vi "UI_Header_Layout.vi"(11 "error in":errorcluster) -> (4 "Specs":T1(array[cluster]), 15 "error out":errorcluster)   [LabVIEW 2026]
doc: "상단 버튼: 0 설정, 1 측정 시작, 2 측정 정지, 3 데이터 저장(저장 중이면 빨강), 4 그래프 창, 5 종료."
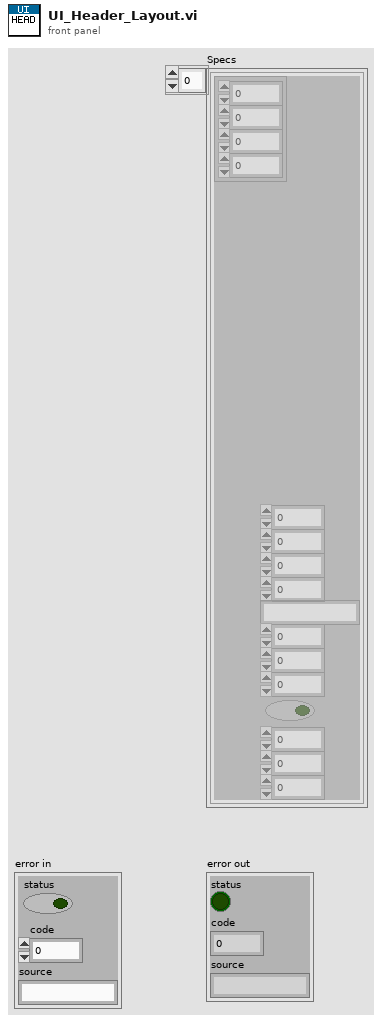
[diagram p1: front panel]
types:
  T1 = cluster{"Rect":cluster{"left":i16, "top":i16, "right":i16, "bottom":i16}, "Fill":u32, "Fill Sel":u32, "Border":u32, "Border Sel":u32, "Text":string, "Text Color":u32, "Text Sel":u32, "Size":i16, "Bold":bool, "Group":i32, "Value":i32, "Radius":i16}[]
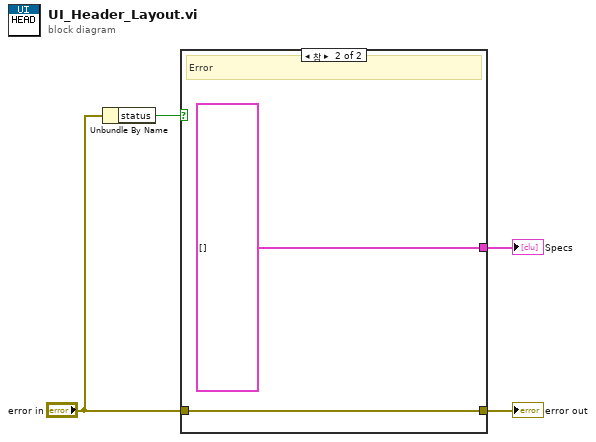
[diagram p0: block diagram]
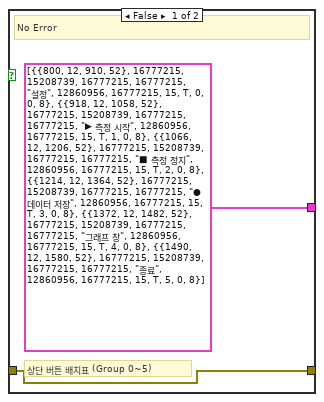
[diagram p2: hidden frame]
diagram:
  n1 = Unbundle By Name("error in") -> ("status"=w2:bool)
  n2 = case shown="참" w2 {
    tunnel: "error in" -> [w5 w7]
    tunnel: [T1 [{"Rect"={"left"=800, "top"=12, "right"=910, "bottom"=52}, "Fill"=16777215, "Fill Sel"=15208739, "Border"=16777215, "Border Sel"=16777215, "Text"="설정", "Text Color"=12860956, "Text Sel"=16777215, "Size"=15, "Bold"=TRUE, "Group"=0, "Value"=0, "Radius"=8}, {"Rect"={"left"=918, "top"=12, "right"=1058, "bottom"=52}, "Fill"=16777215, "Fill Sel"=15208739, "Border"=16777215, "Border Sel"=16777215, "Text"="▶ 측정 시작", "Text Color"=12860956, "Text Sel"=16777215, "Size"=15, "Bold"=TRUE, "Group"=1, "Value"=0, "Radius"=8}, {"Rect"={"left"=1066, "top"=12, "right"=1206, "bottom"=52}, "Fill"=16777215, "Fill Sel"=15208739, "Border"=16777215, "Border Sel"=16777215, "Text"="■ 측정 정지", "Text Color"=12860956, "Text Sel"=16777215, "Size"=15, "Bold"=TRUE, "Group"=2, "Value"=0, "Radius"=8}, {"Rect"={"left"=1214, "top"=12, "right"=1364, "bottom"=52}, "Fill"=16777215, "Fill Sel"=15208739, "Border"=16777215, "Border Sel"=16777215, "Text"="● 데이터 저장", "Text Color"=12860956, "Text Sel"=16777215, "Size"=15, "Bold"=TRUE, "Group"=3, "Value"=0, "Radius"=8}, {"Rect"={"left"=1372, "top"=12, "right"=1482, "bottom"=52}, "Fill"=16777215, "Fill Sel"=15208739, "Border"=16777215, "Border Sel"=16777215, "Text"="그래프 창", "Text Color"=12860956, "Text Sel"=16777215, "Size"=15, "Bold"=TRUE, "Group"=4, "Value"=0, "Radius"=8}, {"Rect"={"left"=1490, "top"=12, "right"=1580, "bottom"=52}, "Fill"=16777215, "Fill Sel"=15208739, "Border"=16777215, "Border Sel"=16777215, "Text"="종료", "Text Color"=12860956, "Text Sel"=16777215, "Size"=15, "Bold"=TRUE, "Group"=5, "Value"=0, "Radius"=8}] ("Header Buttons") T1 []] -> w3
    tunnel: [w5 w7] -> w4
    frame False {
      # "상단 버튼 배치표 (Group 0~5)"
      # "No Error"
    }
    frame True {
      # "Error"
    }
  }
  "Specs" <- w3
  "error out" <- w4
